vi "PicoScope3000aExampleBlockAdvancedTrig.vi"() -> ()   [LabVIEW 2010]
uses:
  shared/PicoBuffers.ctl
  <vilib>/Waveform/DWDTOps.llb/DWDT Analog to Digital.vi
  shared/Buffer and Transfer Settings.ctl
  shared/Acquisition Settings.ctl
  PicoScope3000aLib/PicoScope3000aDigitalChannelSettings.ctl
  PicoScope3000aLib/PicoScope3000aAnalogChannelSettings.ctl
panel:
  in  "Channel B Trigger Properties":T1={"thresholdUpper"=0, "thresholdUpperHysteresis"=1024, "thresholdLower"=0, "thresholdLowerHysteresis"=1024, "Threshold Mode"=0, "Direction"=2, "Available"=FALSE} {"Direction" items=["Above / Inside", "Below / Outside", "Rising / Enter", "Falling / Exit", "Rising or Falling / Enter or Exit", "Above Lower", "Below Lower", "Rising Lower", "Falling Lower", "Positive Runt", "Negative Runt"]; "Threshold Mode" items=["Level", "Window"]}
  in  "Channel B Settings":T2={"Enabled"=FALSE, "Coupling"=1, "Range"=6, "Analogue Offset"=0.0, "Bandwidth Limit"=0} {"Bandwidth Limit" items=["Full", "20MHz"]; "Range" items=["10 mV", "20 mV", "50 mV", "100 mV", "200 mV", "500 mV", "1 V", "2 V", "5 V", "10 V", "20 V", "50 V ", "100 V"]; "Coupling" items=["AC", "DC"]}
  in  "Pulse Width Qualifier Conditions":T3 {"Condition Logic" items=["AND", "OR", "XOR"]}
  in  "Pulse Width Qualifier Settings":T4={"Direction"=2, "Lower Limit"=0, "Upper Limit"=0, "Pulse Width Type"=0} {"Pulse Width Type" items=["None", "Less Than", "Greater Than", "In Range", "Out of Range"]; "Direction" items=["Rising"=2, "Falling"=3]}
  in  "Auto Trigger (ms)":i32=1000
  in  "Trigger Conditions":T5 {"Condition Logic" items=["AND", "OR", "XOR"]}
  in  "Channel A Trigger Properties":T1={"thresholdUpper"=0, "thresholdUpperHysteresis"=1024, "thresholdLower"=0, "thresholdLowerHysteresis"=1024, "Threshold Mode"=0, "Direction"=2, "Available"=FALSE} {"Direction" items=["Above / Inside", "Below / Outside", "Rising / Enter", "Falling / Exit", "Rising or Falling / Enter or Exit", "Above Lower", "Below Lower", "Rising Lower", "Falling Lower", "Positive Runt", "Negative Runt"]; "Threshold Mode" items=["Level", "Window"]}
  in  "Digital Port  0":T6 {"Direction Channel 7" items=["Don't Care", "Low", "High", "Rising", "Falling"]; "Direction Channel 6" items=["Don't Care", "Low", "High", "Rising", "Falling"]; "Direction Channel 5" items=["Don't Care", "Low", "High", "Rising", "Falling"]; "Direction Channel 4" items=["Don't Care", "Low", "High", "Rising", "Falling"]; "Direction Channel 3" items=["Don't Care", "Low", "High", "Rising", "Falling"]; "Direction Channel 2" items=["Don't Care", "Low", "High", "Rising", "Falling"]; "Direction Channel 1" items=["Don't Care", "Low", "High", "Rising", "Falling"]; "Direction Channel 0" items=["Don't Care", "Low", "High", "Rising", "Falling"]}
  in  "Channel A Settings":T2={"Enabled"=TRUE, "Coupling"=1, "Range"=6, "Analogue Offset"=0.0, "Bandwidth Limit"=0} {"Bandwidth Limit" items=["Full", "20MHz"]; "Range" items=["10 mV", "20 mV", "50 mV", "100 mV", "200 mV", "500 mV", "1 V", "2 V", "5 V", "10 V", "20 V", "50 V ", "100 V"]; "Coupling" items=["AC", "DC"]}
  in  "Port 0 Settings":T7={"Enabled"=FALSE, "Logic Level"=9830} {"Logic Level" items=["1.5V TTL"=9830, "2.5V CMOS"=16383]}
  out "overflow":i16 format="%010b"
  in  "Apply Settings":bool
  out "USB 3.0 device on non-USB 3.0 Port":bool=TRUE
  out "USB Powered":bool=TRUE
  out "Device Info":T8={"Driver Version"="2.1.104.3324", "USB Version"="2.0", "Hardware"="1", "Variant"="5244A", "Batch and Serial"="CQ178/007", "Cal Date"="11Jun13", "Kernel Version"="1.0", "Digital HW Version"="1", "Analogue HW Version"="1", "MSO"=FALSE, "Number of channels"=2}
  out "error out":errorcluster
  in  "Data file":path=path "PicoScope3000aExampleBlock ChA Data"
  in  "Buffer and Transfer Settings":T9={"startIndex"=0, "Samples"=5000000, "Down Sample Ratio"=1, "Down-Sample Mode"=0} {"Down-Sample Mode" items=["RAW none"=2147483648, "None"=0, "Aggregate"=1, "Decimate"=2, "Average"=4]; "Down Sample Ratio" step=1; "Samples" format="%_6p"}
  in  "Acquisition Settings":T10={"preTriggerSamples"=0, "postTriggerSamples"=5000000, "timebase"=5} {"postTriggerSamples" format="%_6p"; "preTriggerSamples" format="%_6p"}
  out "Properties Panel":T11={"Sample Frequency"=41666668.0, "Sample Rate"=2.4000000209412065e-08, "Max Samples Available"=26843008, "Number of Samples"=0, "Total Capture Time (sec) "=0.0, "Max Total Capture Time Available (sec)"=0.6442322134971619} {"Max Total Capture Time Available (sec)" format="%.3p"; "Sample Frequency" format="%.6p"; "Sample Rate" format="%.3p"; "Max Samples Available" format="%_6p"; "Total Capture Time (sec)" format="%.3p"}
  out "Port 0":digitalwaveform(graph)={"t0"=timestamp(0 s since 1904-01-01), "dt"=8e-09, "Y"={"transitions"=[], "data"=[]}}
  in  "stop":bool
  out "Analog Channels":cluster{i32, sgl, "Data":dbl[]}[](graph)
  in  "Serial Number":string
  in  "Use Serial Number":bool
  in  "error in (no error)":errorcluster
  # "Bit 0 = ChA"
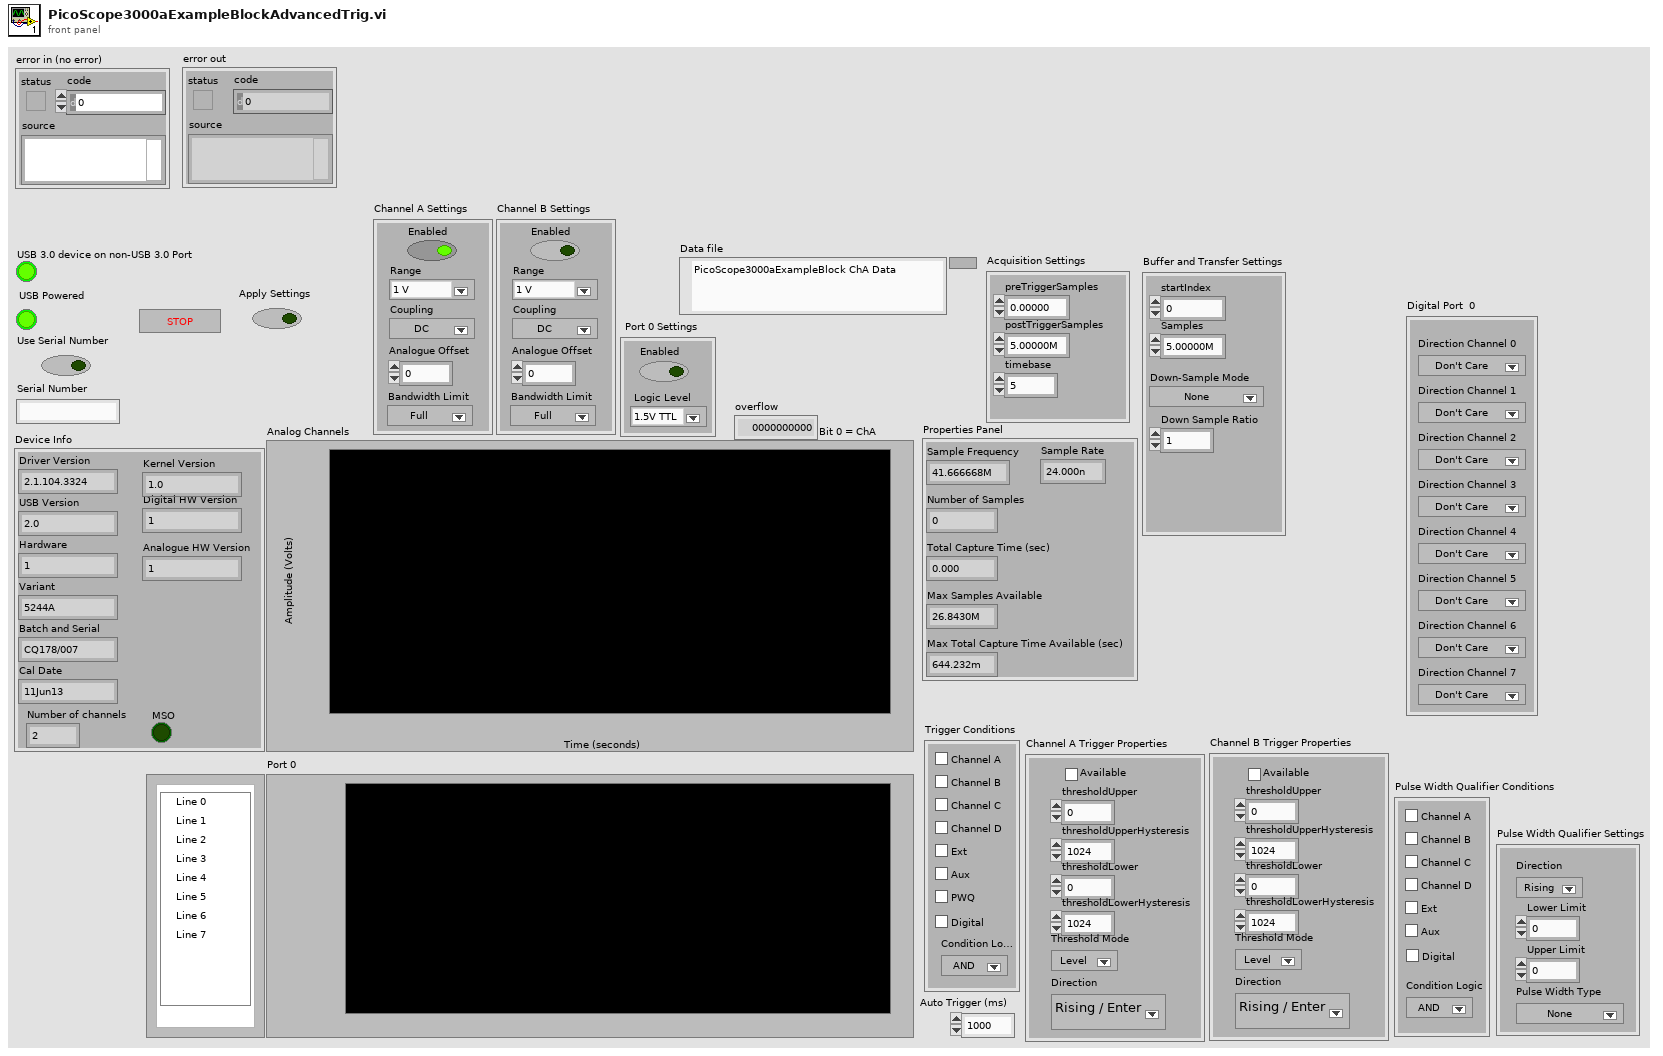
[diagram p1: front panel]
types:
  T1 = cluster{"thresholdUpper":i16, "thresholdUpperHysteresis":u16, "thresholdLower":i16, "thresholdLowerHysteresis":u16, "Threshold Mode":i32, "Direction":i32, "Available":bool}
  T2 = typedef "PicoScope3000aAnalogChannelSettings.ctl" = cluster{"Enabled":bool, "Coupling":u32, "Range":u32, "Analogue Offset":sgl, "Bandwidth Limit":u32}
  T3 = cluster{"Channel A":bool, "Channel B":bool, "Channel C":bool, "Channel D":bool, "Aux":bool, "Condition Logic":u16, "Ext":bool, "Digital":bool}
  T4 = cluster{"Direction":u32, "Lower Limit":u32, "Upper Limit":u32, "Pulse Width Type":u32}
  T5 = cluster{"Channel A":bool, "Channel B":bool, "Channel C":bool, "Channel D":bool, "Aux":bool, "PWQ":bool, "Condition Logic":u16, "Ext":bool, "Digital":bool}
  T6 = cluster{"Direction Channel 0":u16, "Direction Channel 1":u16, "Direction Channel 2":u16, "Direction Channel 3":u16, "Direction Channel 4":u16, "Direction Channel 5":u16, "Direction Channel 6":u16, "Direction Channel 7":u16}
  T7 = typedef "PicoScope3000aDigitalChannelSettings.ctl" = cluster{"Enabled":bool, "Logic Level":i16}
  T8 = cluster{"Driver Version":string, "USB Version":string, "Hardware":string, "Variant":string, "Batch and Serial":string, "Cal Date":string, "Kernel Version":string, "Digital HW Version":string, "Analogue HW Version":string, "MSO":bool, "Number of channels":i16}
  T9 = typedef "Buffer and Transfer Settings.ctl" = cluster{"startIndex":u64, "Samples":u64, "Down Sample Ratio":u64, "Down-Sample Mode":u32}
  T10 = typedef "Acquisition Settings.ctl" = cluster{"preTriggerSamples":u64, "postTriggerSamples":u64, "timebase":u32}
  T11 = cluster{"Sample Frequency":dbl, "Sample Rate":dbl, "Max Samples Available":u64, "Number of Samples":u64, "Total Capture Time (sec) ":dbl, "Max Total Capture Time Available (sec)":dbl}
  T12 = enum16{"open", "open or create", "create or replace", "create", "open (read-only)"}
  T13 = typedef "PicoBuffers.ctl" = cluster{"Max Buffer Pointers":u64[][][], "Min Buffer Pointers":u64[][][], "StreamingDataInfo":cluster{"Channel":u32, "Down-Sample Mode":u32, "PICO_DATA_TYPE":enum32{"PICO_INT8_T", "PICO_INT16_T", "PICO_INT32_T", "PICO_UINT32_T", "PICO_INT64_T", ""}, "Samples":i32, "bufferIndex":u64, "startIndex":i32, "overflow":i16}[][]}
  T14 = cluster{"Sample Frequency":sgl, "Sample Rate":sgl, "Max Samples Available":i32, "Number of Samples":u32, "Total Capture Time (sec) ":sgl, "Max Total Capture Time Available (sec)":sgl}
  T15 = cluster{"Channel A Buffer":i16[], "Channel B Buffer":i16[], "Channel C Buffer":i16[], "Channel D Buffer":i16[], "Channel E Buffer":i16[], "Channel F Buffer":i16[], "Channel G Buffer":i16[], "Channel H Buffer":i16[], "Port 0 Buffer":i16[], "Port 1 Buffer":i16[]}[]
  T16 = cluster{"Channel A Buffer":i16[], "Channel B Buffer":i16[], "Channel C Buffer":i16[], "Channel D Buffer":i16[], "Channel E Buffer":i16[], "Channel F Buffer":i16[], "Channel G Buffer":i16[], "Channel H Buffer":i16[], "Port 0 Buffer":i16[], "Port 1 Buffer":i16[]}
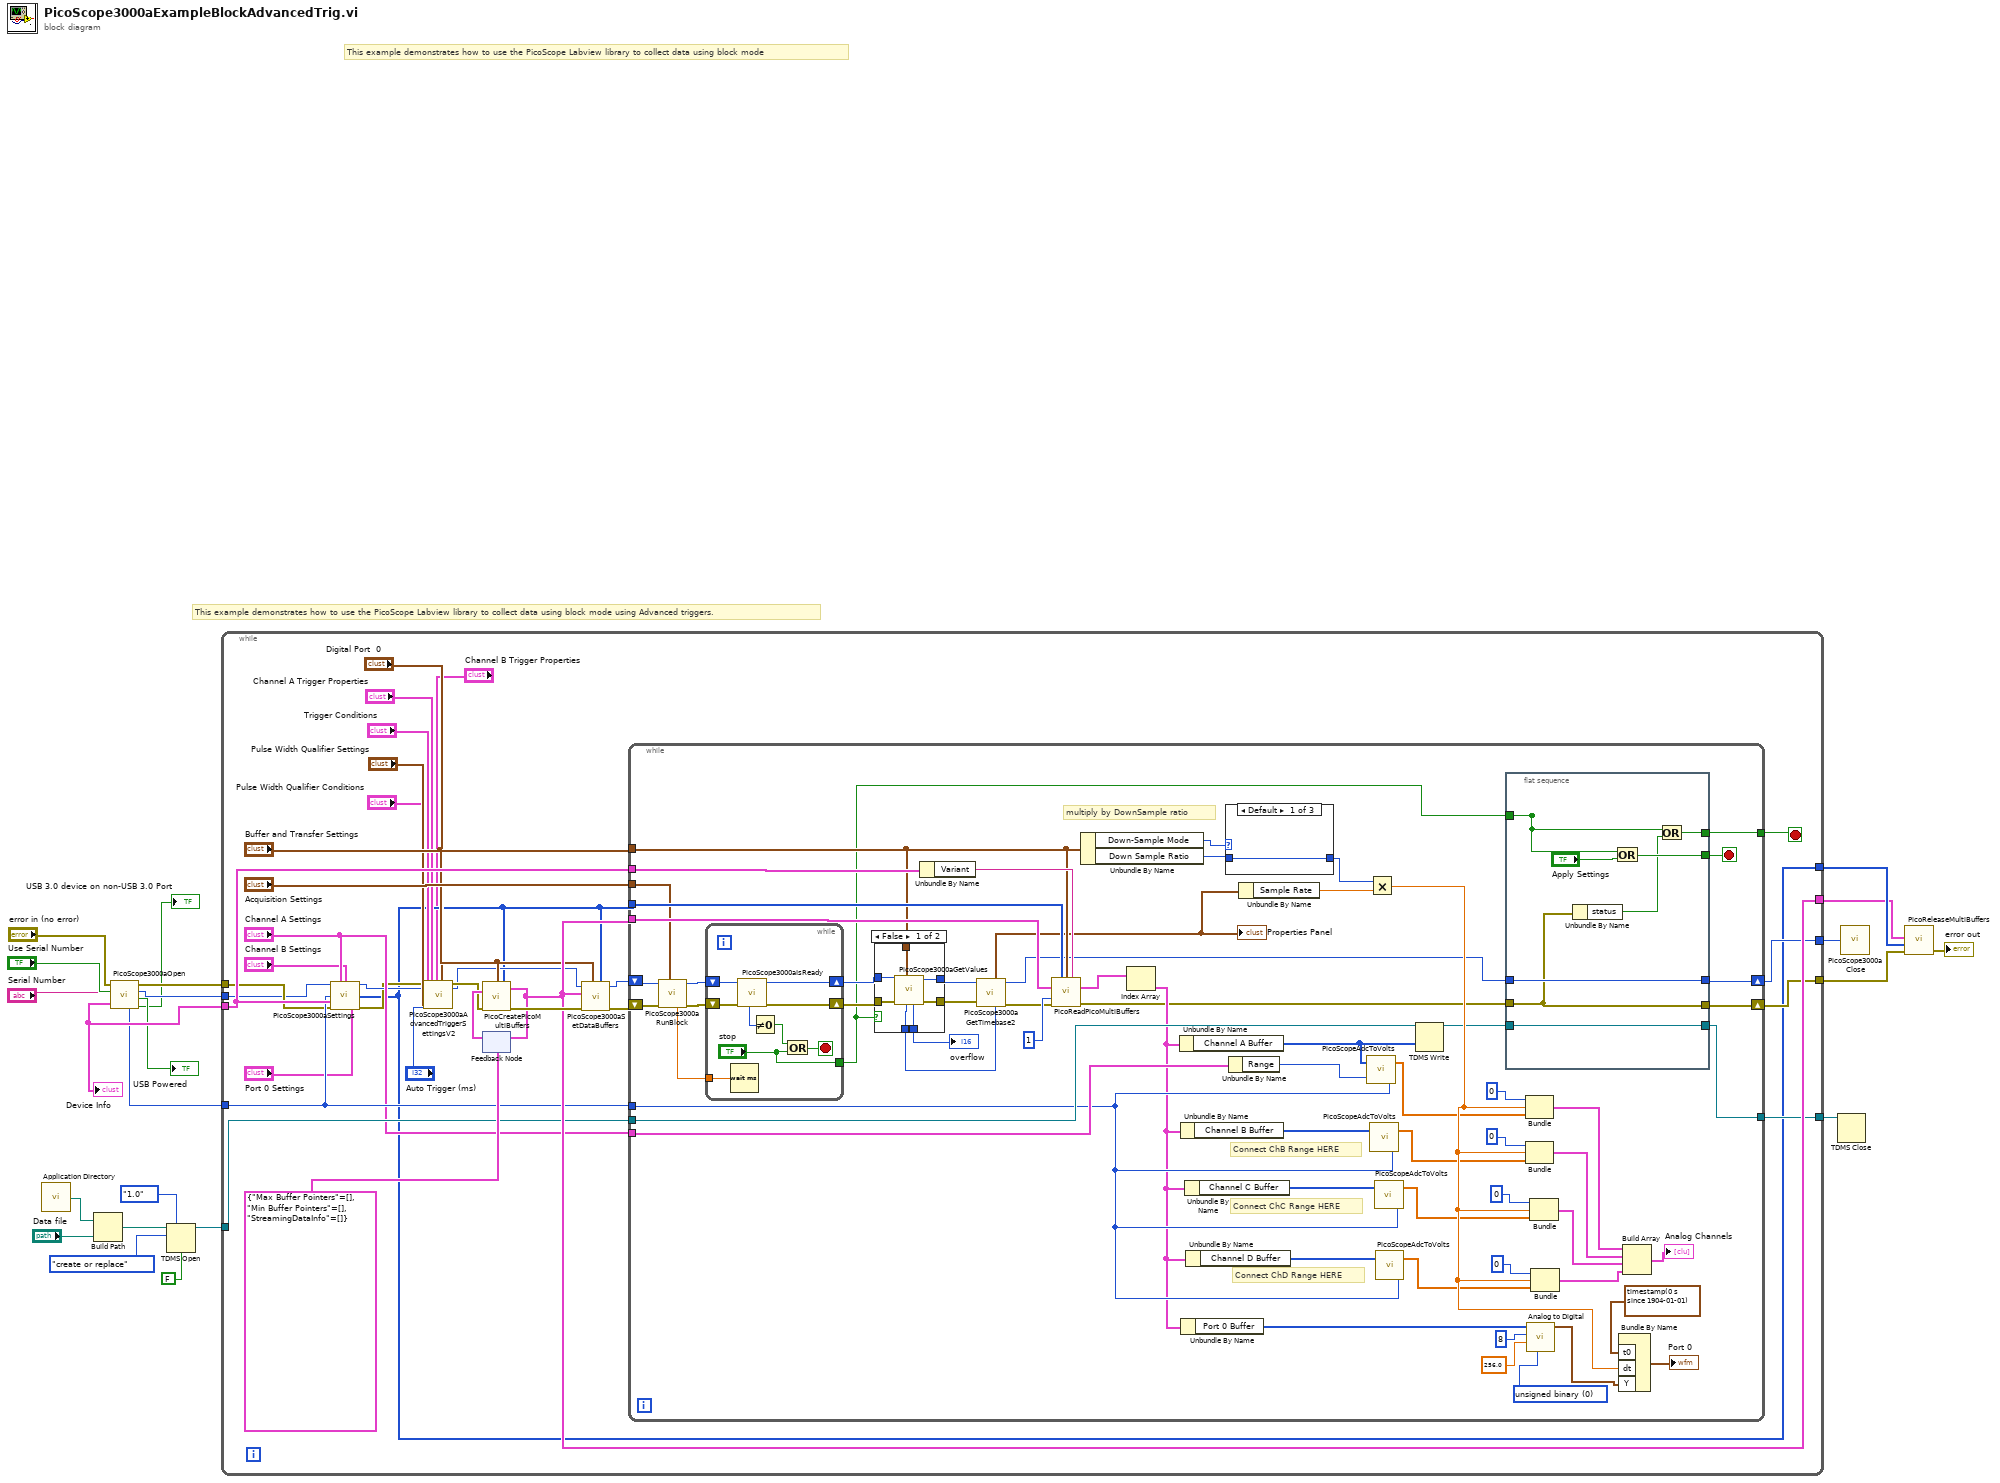
[diagram p0: block diagram]
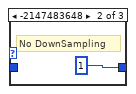
[diagram p3: hidden frame]
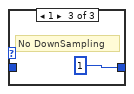
[diagram p4: hidden frame]
diagram:
  # "This example demonstrates how to use the PicoScope Labview library to collect data using block mode using Advanced triggers."
  # "This example demonstrates how to use the PicoScope Labview library to collect data using block mode"
  n1 = call <vilib>:"Application Directory.vi"() -> ("Application Directory"=w14:path)
  n2 = Build Path(base path=w14, name or relative path="Data file") -> (appended path=w15:path)
  n3 = call "PicoScope3000aOpen.vi"("Batch/Serial"="Serial Number", "Use Serial number"="Use Serial Number", "error in (no error)"="error in (no error)") -> ("USB 3.0 device on non-USB 3.0 Port"=→"USB 3.0 device on non-USB 3.0 Port":bool, "USB Powered"=→"USB Powered":bool, "handle"=w22:i16, "error out"=w5:errorcluster, "Max ADC value"=w2:i16, "Device Info"=w7:T8)  [unwired: 3 in]
  "Device Info" <- w7
  n4 = TDMS Open(6:FALSE ("disable buffering? (T)"), 7:enum16{"1.0", "2.0"}."1.0" ("file format version (2.0)"), 10:T12."create or replace" ("operation (0:open)"), 11:w15) -> (3:w12:refnum<k34>)  [unwired: 2 in, 1 out]
  n5 = while {
    tunnel: w22 -> [w28]
    tunnel: w2 -> [w40]
    tunnel: [w25] -> w21
    tunnel: [w51] -> w20
    tunnel: [w46] -> w13
    tunnel: w12 -> [w50]
    tunnel: w7 -> [w48]
    tunnel: w5 -> [w29]
    tunnel: [w47] -> w4
    tunnel: [w44] -> w3
    stop <- w45 stop-if-true
    n6 = call "PicoScope3000aSettings.vi"("handle in"=w28, "Channel A Settings"="Channel A Settings", "Channel B Settings"="Channel B Settings", "Port 0 Settings"="Port 0 Settings", "Max_adc"=w40, "Device Info"=w48, "error in"=w29) -> ("handle out"=w27:i16, "Enabled Array"=w25:i16[], "error out"=w26:errorcluster)  [unwired: 6 in]
    n7 = call "PicoScope3000aAdvancedTriggerSettingsV2.vi"("error in"=w26, "handle in"=w27, "Trigger Conditions"="Trigger Conditions", "Auto Trigger (ms)"="Auto Trigger (ms)", "Channel A Trigger Properties"="Channel A Trigger Properties", "Channel B Trigger Properties"="Channel B Trigger Properties", "Digital Port  0"="Digital Port  0", "Pulse Width Qualifier Conditions"="Pulse Width Qualifier Conditions", "Pulse Width Qualifier Settings"="Pulse Width Qualifier Settings") -> ("error out"=w37:errorcluster, "handle out"=w36:i16)  [unwired: 9 in]
    n8 = feedback #1(T13 {"Max Buffer Pointers"=[], "Min Buffer Pointers"=[], "StreamingDataInfo"=[]} ("Data Pointers")) -> (w53:T13)
    n9 = call "PicoCreatePicoMultiBuffers.vi"("Buffer and Transfer Settings"="Buffer and Transfer Settings", "enabled array"=w25, "Data Pointers In"=w53, "error in (no error)"=w37) -> ("Data Pointers"=w51:T13, "error out"=w52:errorcluster)  [unwired: 10 in]
    n10 = feedback-in #1(w51) -> ()
    n11 = call "PicoScope3000aSetDataBuffers.vi"("enabled array"=w25, "Buffer and Transfer Settings"="Buffer and Transfer Settings", "error in (no error)"=w52, "Data Pointers In"=w51, "handle in"=w36) -> ("error out"=w43:errorcluster, "handle out"=w42:i16)  [unwired: 5 in]
    n12 = while {
      tunnel: w51 -> [w118]
      tunnel: "Buffer and Transfer Settings" -> [w63]
      tunnel: w25 -> [w109]
      tunnel: "Channel A Settings" -> [w108]
      tunnel: "Acquisition Settings" -> [w107]
      tunnel: w40 -> [w106]
      tunnel: w48 -> [w103]
      tunnel: [w70] -> w45
      shift-right: [w74] -> w47
      shift-left: w43 -> [w64]
      shift-right: [w68] -> w44
      shift-left: w42 -> [w65]
      tunnel: w50 -> [w117]
      tunnel: [w72] -> w46
      stop <- w69 stop-if-true
      w91 = u16 0 items=["unsigned binary", "offset binary", "2's complement"] ("data format (offset binary)")
      # "Connect ChB Range HERE"
      # "Connect ChD Range HERE"
      # "Connect ChC Range HERE"
      # "multiply by DownSample ratio"
      n13 = call "PicoScope3000aRunBlock.vi"("Acquisition Settings"=w107, "error in (no error)"=w64, "handle in"=w65) -> ("error out"=w111:errorcluster, "handle out"=w110:i16, "timeIndisposedMs"=w101:dbl)  [unwired: 5 in, 1 out]
      n14 = while {
        shift-right: [w143] -> w66
        shift-left: w111 -> [w144]
        shift-right: [w142] -> w67
        shift-left: w110 -> [w141]
        tunnel: ["stop"] -> w62
        tunnel: w101 -> [w136]
        stop <- w138 stop-if-true
        n15 = Wait (ms)(milliseconds to wait=w136) -> ()  [unwired: 1 out]
        n16 = call "PicoScope3000aIsReady.vi"("error in (no error)"=w144, "handle in"=w141) -> ("error out"=w143:errorcluster, "handle out"=w142:i16, "ready"=w140:i16)  [unwired: 7 in]
        n17 = Not Equal To 0?(x=w140) -> (x != 0?=w139:bool)
        n18 = Or(x=w139, y="stop") -> (x .or. y?=w138:bool)
      }
      n19 = case shown="False" w62 {
        tunnel: w66 -> [w125 w126]
        tunnel: w67 -> [w124 w127]
        tunnel: [w123 w127] -> w57
        tunnel: [w122 w126] -> w58
        tunnel: w63 -> [w121 _]
        tunnel: [w120 _] -> w61
        tunnel: [w119 _] -> w60
        frame False {
          n20 = call "PicoScope3000aGetValues.vi"("Buffer and Transfer Settings"=w121, "error in (no error)"=w125, "handle in"=w124) -> ("error out"=w122:errorcluster, "handle out"=w123:i16, "overflow"=w120:i16, "noOfSamples"=w119:u64)  [unwired: 5 in]
        }
        frame True {
        }
      }
      "overflow" <- w61
      n21 = Unbundle By Name(w103) -> ("Variant"=w104:string)
      n22 = call "PicoScope3000aGetTimebase2.vi"("Number of Samples"=w60, "error in (no error)"=w58, "handle in"=w57) -> ("error out"=w56:errorcluster, "handle out"=w55:i16, "Properties Panel"=w59:T14)  [unwired: 6 in]
      "Properties Panel" <- w59
      n23 = call "PicoReadPicoMultiBuffers.vi"("enabled array"=w109, "Buffer and Transfer Settings"=w63, "Variant"=w104, "Data Pointers"=w118, "No of Buffers"=1, "error in (no error)"=w56) -> ("MultiBuffers (Max or non-aggregated)"=w116:T15, "error out"=w71:errorcluster)  [unwired: 7 in, 1 out]
      n24 = Unbundle By Name(w63) -> ("Down-Sample Mode"=w114:u32, "Down Sample Ratio"=w115:u64)
      n25 = Index Array(array=w116) -> (element=w75:T16)  [unwired: 1 in]
      n26 = Unbundle By Name(w75) -> ("Channel A Buffer"=w84:i16[])
      n27 = Unbundle By Name(w75) -> ("Channel B Buffer"=w97:i16[])
      n28 = Unbundle By Name(w75) -> ("Port 0 Buffer"=w89:i16[])
      n29 = Unbundle By Name(w75) -> ("Channel C Buffer"=w82:i16[])
      n30 = Unbundle By Name(w75) -> ("Channel D Buffer"=w78:i16[])
      n31 = case shown="Default" w114 {
        tunnel: [w145 u64 1 ("Down Sample Ratio") u64 1 ("Down Sample Ratio")] -> w112
        tunnel: w115 -> [w145 _ _]
        frame Default {
        }
        frame -2147483648 {
          # "No DownSampling"
        }
        frame 1 {
          # "No DownSampling"
        }
      }
      n32 = Unbundle By Name(w108) -> ("Range"=w99:u32)
      n33 = Unbundle By Name(w59) -> ("Sample Rate"=w105:sgl)
      n34 = call "PicoScopeAdcToVolts.vi"("Max_adc"=w106, "Range Index"=w99, "Data"=w84) -> ("Data"=w85:dbl[])
      n35 = Multiply(x=w112, y=w105) -> (x*y=w113:sgl)
      n36 = call "PicoScopeAdcToVolts.vi"("Max_adc"=w106, "Data"=w97) -> ("Data"=w96:dbl[])  [unwired: 1 in]
      n37 = call "PicoScopeAdcToVolts.vi"("Max_adc"=w106, "Data"=w82) -> ("Data"=w81:dbl[])  [unwired: 1 in]
      n38 = call "PicoScopeAdcToVolts.vi"("Max_adc"=w106, "Data"=w78) -> ("Data"=w77:dbl[])  [unwired: 1 in]
      n39 = TDMS Write(0:w117, 9:w84) -> (4:w73:refnum<k34>)  [unwired: 4 in, 3 out]
      n40 = flat-sequence {
        tunnel: [w135] -> w69
        tunnel: [w128] -> _
        tunnel: [w132] -> w70
        tunnel: w55 -> [w131]
        tunnel: [w131] -> w68
        tunnel: w71 -> [w130]
        tunnel: [w130] -> w74
        tunnel: [w129] -> w72
        tunnel: w73 -> [w129]
        tunnel: w62 -> [w128]
        frame #0 {
          n41 = Unbundle By Name(w130) -> ("status"=w133:bool)
          n42 = Or(x=w128, y="Apply Settings") -> (x .or. y?=w135:bool)
          n43 = Or(x=w128, y=w133) -> (x .or. y?=w132:bool)
        }
      }
      n44 = Bundle(0, w113, "Data"=w85) -> (w95:cluster{i32, sgl, "Data":dbl[]})  [unwired: 1 in]
      n45 = Bundle(0, w113, "Data"=w96) -> (w94:cluster{i32, sgl, "Data":dbl[]})  [unwired: 1 in]
      n46 = call-poly <vilib>:"Analog to Digital.vi"("data format (offset binary)"=w91, "full-scale range (pk-pk)"=256.0, "resolution (16 bit)"=8, "analog waveform"=w89) -> ("digital waveform"=w86:digitalwaveform)  [unwired: 4 in, 3 out]
      n47 = Bundle(0, w113, "Data"=w81) -> (w80:cluster{i32, sgl, "Data":dbl[]})  [unwired: 1 in]
      n48 = Bundle(0, w113, "Data"=w77) -> (w76:cluster{i32, sgl, "Data":dbl[]})  [unwired: 1 in]
      n49 = Bundle By Name("t0"=timestamp(0 s since 1904-01-01), "dt"=w113, "Y"=w86) -> (→"Port 0":digitalwaveform)  [unwired: 1 in]
      n50 = Build Array(w95, w94, w80, w76) -> (→"Analog Channels":cluster{i32, sgl, "Data":dbl[]}[])
    }
  }
  n51 = TDMS Close(11:w13) -> ()  [unwired: 1 in, 2 out]
  n52 = call "PicoScope3000aClose.vi"("handle"=w3) -> ()
  n53 = call "PicoReleaseMultiBuffers.vi"("error in (no error)"=w4, "Enabled array"=w21, "Data Pointers"=w20) -> ("error out"=→"error out":errorcluster)  [unwired: 8 in]
